vi "SeqEditor_DATASAVE.vi"(8 "error in (no error)":errorcluster, 11 "NLTest in":refnum<class "NLTest.lvclass">) -> (0 "error out":errorcluster, 3 "NLTest out":refnum<class "NLTest.lvclass">)   [LabVIEW 2017, in "NLTest.lvclass"]
uses:
  NLTest.lvclass
  NLTest.lvclass/NLTest.ctl
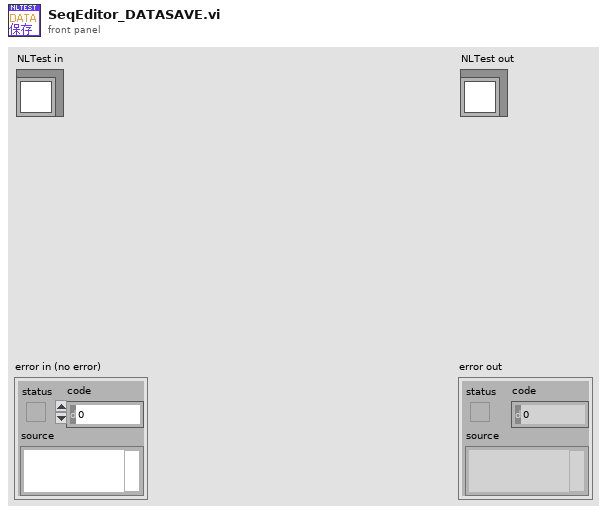
[diagram p1: front panel]
types:
  T1 = enum16{"open", "replace", "create", "open or create", "replace or create", "replace or create with confirmation"}
  T2 = typedef "NLTest.lvclass/allseqanddata.ctl" = cluster{"seqname":string, "seqdata":string[]}
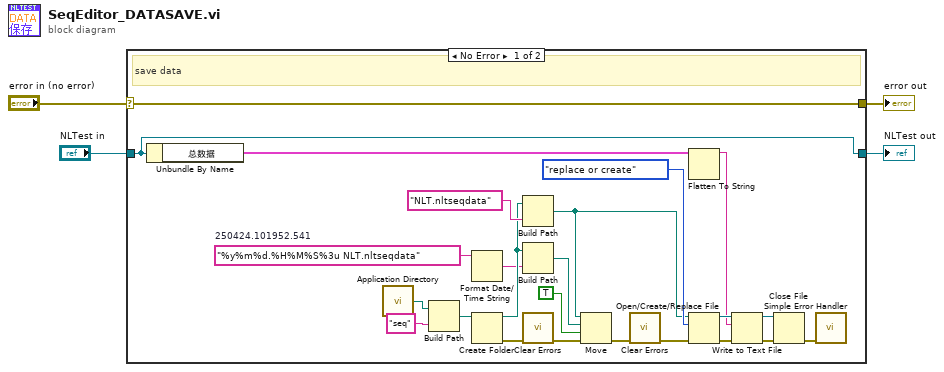
[diagram p0: block diagram]
diagram:
  n1 = case shown="No Error" "error in (no error)" {
    selector: "error in (no error)" -> [w28 w30]
    tunnel: [w28 w30] -> w3
    tunnel: [w15 w29] -> w1
    tunnel: "NLTest in" -> [w15 w29]
    frame No Error {
      w8 = "%y%m%d.%H%M%S%3u NLT.nltseqdata"  # 250424.101952.541
      # "save data"
      n2 = Unbundle By Name(w15) -> ("总数据"=w16:T2[])
      n3 = call <vilib>:"Application Directory.vi"() -> ("Application Directory"=w27:path)
      n4 = Build Path(base path=w27, name or relative path="seq") -> (appended path=w26:path)
      n5 = Format Date/Time String(time format string (%c)=w8) -> (date/time string=w7:string)  [unwired: 2 in]
      n6 = Create Folder(path (use dialog)=w26) -> (created path=w11:path, error out=w24:errorcluster)  [unwired: 2 in, 1 out]
      n7 = Build Path(base path=w11, name or relative path="NLT.nltseqdata") -> (appended path=w12:path)
      n8 = Build Path(base path=w11, name or relative path=w7) -> (appended path=w10:path)
      n9 = call <vilib>:"Clear Errors.vi"("error in (no error)"=w24) -> ("error out"=w13:errorcluster)  [unwired: 5 in, 1 out]
      n10 = Move(source path=w12, error in=w13, 9:TRUE ("overwrite (F)"), 10:w10) -> (error out=w6:errorcluster)  [unwired: 1 in, 2 out]
      n11 = call <vilib>:"Clear Errors.vi"("error in (no error)"=w6) -> ("error out"=w5:errorcluster)  [unwired: 5 in, 1 out]
      n12 = Flatten To String(anything=w16) -> (data string=w14:string)  [unwired: 3 in, 2 out]
      n13 = Open/Create/Replace File(file path (use dialog)=w12, error in=w5, operation (0:open)=T1."replace or create") -> (refnum out=w20:refnum<file>, error out=w21:errorcluster)  [unwired: 3 in, 1 out]
      n14 = Write to Text File(file (use dialog)=w20, text=w14, error in=w21) -> (refnum out=w18:refnum<file>, error out=w19:errorcluster)  [unwired: 1 in, 1 out]
      n15 = Close File(refnum=w18, error in=w19) -> (error out=w17:errorcluster)  [unwired: 1 out]
      n16 = call <vilib>:"Simple Error Handler.vi"("error in (no error)"=w17) -> ()  [unwired: 4 in, 5 out]
    }
    frame Error {
    }
  }
  "error out" <- w3
  "NLTest out" <- w1
